vi "FluidtekPrensaCONidentLEDI_v16.vi"() -> ()   [LabVIEW 2026]
uses:
  <vilib>/DAQmx/read.llb/DAQmx Read (Digital 1D Bool NChan 1Samp 1Line).vi
  <vilib>/DAQmx/write.llb/DAQmx Write (Digital 1D Bool NChan 1Samp 1Line).vi
  <vilib>/DAQmx/read.llb/DAQmx Read (Analog 1D Wfm NChan NSamp).vi
  <vilib>/Analysis/baseanly.llb/Mean (DBL).vi
  <vilib>/DAQmx/write.llb/DAQmx Write (Analog DBL 1Chan 1Samp).vi
  <extravilib>/ChannelInstances/Tag-bool/Read With Abort.vi
  <extravilib>/ChannelInstances/Tag-c(dbl,dbl,dbl,dbl,dbl,dbl)/Read With Abort.vi
  <extravilib>/ChannelInstances/Tag-c(dbl,dbl,dbl,dbl,dbl,dbl,dbl,bool,u16)/Write With Abort.vi
  <extravilib>/ChannelInstances/Tag-bool/Write With Abort.vi
  <extravilib>/ChannelInstances/Tag-c(dbl,dbl,dbl,dbl,dbl,dbl,dbl,bool,u16)/Read With Abort.vi
  <extravilib>/ChannelInstances/Tag-c(dbl,dbl,dbl,dbl,dbl,dbl)/Write With Abort.vi
  GlobalesPrensa.vi
  <vilib>/Utility/file.llb/Write Delimited Spreadsheet (DBL).vi
  <vilib>/DAQmx/create/channels.llb/DAQmx Create Channel (AO-Voltage-Basic).vi
  <vilib>/DAQmx/create/channels.llb/DAQmx Create Channel (AI-Voltage-Basic).vi
  <vilib>/DAQmx/configure/timing.llb/DAQmx Timing (Sample Clock).vi
  <vilib>/DAQmx/create/channels.llb/DAQmx Create Channel (DO-Digital Output).vi
  <vilib>/DAQmx/create/channels.llb/DAQmx Create Channel (DI-Digital Input).vi
  <extravilib>/ChannelInstances/Tag-bool/Instantiate.vi
  <extravilib>/ChannelInstances/Tag-bool/Endpoint.vi
  <vilib>/DAQmx/miscellaneous.llb/DAQmx Fill In Error Info.vi
  <extravilib>/ChannelInstances/Tag-c(dbl,dbl,dbl,dbl,dbl,dbl,dbl,bool,u16)/Instantiate.vi
  <extravilib>/ChannelInstances/Tag-c(dbl,dbl,dbl,dbl,dbl,dbl)/Instantiate.vi
  <extravilib>/ChannelInstances/Tag-bool/EndpointRead.vi
  <extravilib>/ChannelInstances/Tag-c(dbl,dbl,dbl,dbl,dbl,dbl)/EndpointRead.vi
  <extravilib>/ChannelInstances/Tag-c(dbl,dbl,dbl,dbl,dbl,dbl,dbl,bool,u16)/Endpoint.vi
  <extravilib>/ChannelInstances/Tag-c(dbl,dbl,dbl,dbl,dbl,dbl,dbl,bool,u16)/EndpointRead.vi
  <extravilib>/ChannelInstances/Tag-c(dbl,dbl,dbl,dbl,dbl,dbl)/Endpoint.vi
  <vilib>/Analysis/NI_AALBase.lvlib
  <extravilib>/ChannelInstances/Tag-bool.lvlib
  <extravilib>/ChannelInstances/Tag-c(dbl,dbl,dbl,dbl,dbl,dbl).lvlib
  <vilib>/ptbypt/NI_PtbyPt.lvlib
  <extravilib>/ChannelInstances/Tag-c(dbl,dbl,dbl,dbl,dbl,dbl,dbl,bool,u16).lvlib
panel:
  out "Archivo":path
  out "Lg log":dbl[](array[numeric])
  in  "PARO DE EMERGENCIA":bool
  out "time/iteration (ms)":u32=210
  in  "Tab Control 3":enum32{"ENSAYO", "REGISTRO"}(tab)
  in  "Tipo ensayos":u16(ring)=1 items=["Flexotraccion en losas", "Tenacidad Vigas"]
  in  "Rampa (mm/min)":dbl=0.1 min=0.0 max=25.0 format="%.3f"
  in  "Rampa (kN/min)":dbl=0.1 min=0.0 max=20.0 format="%.2f"
  in  "Limite fuerza (kN)":dbl=3.0 min=0.0 max=150.0 format="%.2f"
  in  "Limite posicion (mm)":dbl=145.0 min=0.0 max=150.0 format="%.2f"
  in  "Tiempo carga (s)":dbl=3.0 min=0.0 max=300.0 format="%.2g"
  out "Tiempo (s)":dbl format="%.2f"
  in  "Iniciar ensayo":bool
  out "Velocidad norma (mm/min)  2":string="0.05 - 0.1"
  in  "Tenacidad en vigas":u16(ring) items=["ASTM 1609 con100x100x350", "ASTM 1609 con150x150x500", "EFNARC 1996", "VIGAS 14651", "ENS. BARCELONA"]
  in  "Aplicar velocidad de norma":bool
  out "Estado del ensayo":dbl(ring) items=["REPOSO", "CARGA (rampa)", "MANTENIENDO CARGA", "DESCARGA", "RETORNO / FIN", "FALLA - ENSAYO DETENIDO", ""]
  in  "Flexotracción en losas":u16(ring)=3 items=["EFNARC 1996", "EFNARC 1999", "EFNARC 14488-5", "ASTM 1550"]
  out "Velocidad norma (mm/min)":dbl=4.0
  in  "IPAddress QuantumX":string="172.31.236.115"
  out "LicenseIsValid":bool
  in  "Registrar":bool
  in  "ID manual (0=auto)":i32
  in  "Tipo":string
  in  "INFLE":dbl
  in  "Detener registro":bool
  in  "Tab Control 2":T1(tab)
  out "Presión B (bar)":dbl=31.47939829954219 format="%.2f"
  out "Presión A (bar)":dbl=47.7049180327869 format="%.2f"
  out "Vertical Progress Bar":dbl(slide)=3.0
  in  "Tab Control":enum32{"Desplazamiento", "Fuerza"}(tab)
  in  "PID fuerza":T2={"proportional gain (Kc)"=1.0, "integral time (Ti, min)"=0.03, "derivative time (Td, min)"=0.0} {"derivative time (Td, min)" format="%.3f"; "integral time (Ti, min)" format="%.3f"; "proportional gain (Kc)" format="%.3f"}
  out "control signals":dynamicdata(graph)=[{"t0"=timestamp(3594752785.1434503 s since 1904-01-01), "dt"=1.0, "Y"=[3.0]}, {"t0"=timestamp(3594752785.1434503 s since 1904-01-01), "dt"=1.0, "Y"=[3.0680651042487943]}]
  in  "Posicion deseada (mm)":dbl(slide)=3.0 min=2.0 max=150.0 scale format="%#_2f"
  in  "Fuerza deseada (kN)":dbl=0.5 min=0.0 max=150.0 format="%.2f"
  out "Fuerza actual (KN)":dbl format="%.2f"
  out "Posicion actual (mm)":dbl format="%.2f"
  in  "Tipo control":u16(ring) items=["Desplazamiento", "Fuerza"]
  out "fuerza desplazamiento":cluster{dbl[], dbl[]}(graph)
  out "Rigidez estimada (kN/mm)":dbl
  out "Carga maxima (kN)":dbl
  out "Progreso mantenimiento":dbl(slide) scale=0.0..100.0
  out "Tiempo restante carga (s)":dbl
  out "Falla":bool
  out "Causa de la falla":dbl(ring) items=["Sin falla", "CAIDA DE CARGA (rotura)", "SOBRECARGA", "LIMITE DE POSICION", "PARO DE EMERGENCIA", "LIMITE DEL SISTEMA (160 kN)", "SIN LECTURA DE FUERZA (QuantumX)", "LIMITE POR PRESIONES (160 kN)"]
  out "Proteccion de fuerza activa":bool
  in  "Vel. aproximacion (mm/min)":dbl=50.0 min=0.1 max=50.0
  in  "Fmax fuera de ensayo (kN)":dbl=1.0 min=0.2 max=50.0
  out "UPH energizada":bool=TRUE
  out "Nivel tanque":bool
  out "Estado de  filtro":bool=TRUE
  out "Sobrecorriente":bool
  in  "Stop":bool
  out "Estado de motor":bool
  in  "Apagar":bool
  in  "Encender":bool
  in  "Sin proteccion de carga":bool
  out "Consigna posicion interna (mm)":dbl
  out "Parametros avanzados":dbl(ring) items=["POR DEFECTO (bloqueados)", "PERSONALIZADOS (activos)"]
  in  "Codigo acceso":dbl
  in  "Kf lazo fuerza (1/s)":dbl=0.5
  in  "Kx lazo posicion (V/mm)":dbl=30.0
  in  "Ti lazo posicion (s)":dbl=1.5
  # "PB"
  # "PA"
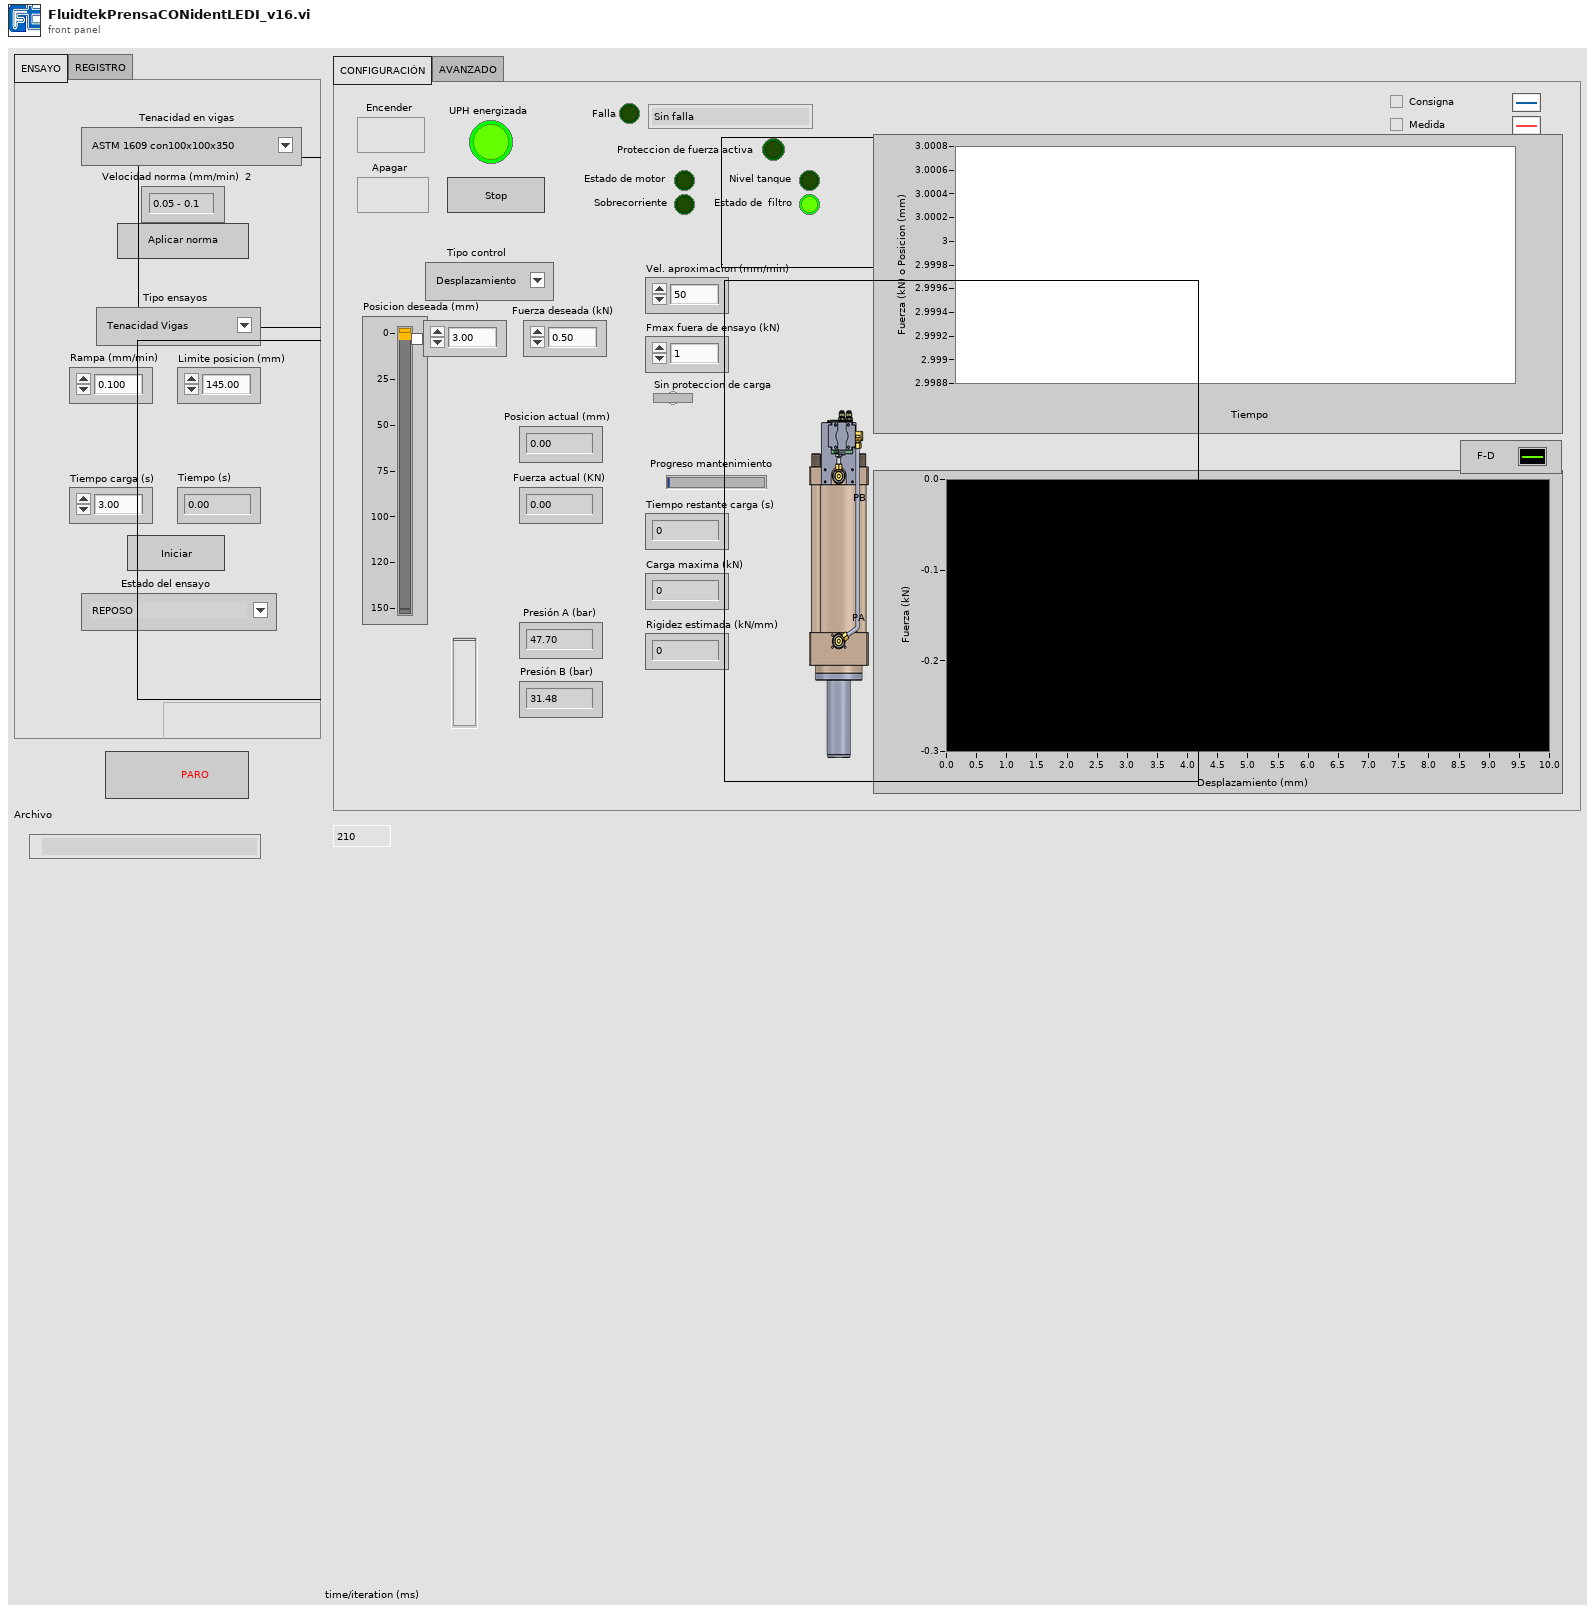
[diagram p1: front panel]
types:
  T1 = enum32{"CONFIGURACIÓN", "AVANZADO", "identificación (no modificar)"}
  T2 = cluster{"proportional gain (Kc)":dbl, "integral time (Ti, min)":dbl, "derivative time (Td, min)":dbl}
  T3 = typedef "Tag-bool.lvlib/))Channel.ctl" = refnum<queue>
  T4 = cluster{"Devices":refnum<k24>[], "Signals":refnum<k24>[]}
  T5 = cluster{"Rampa (mm/min)":dbl, "Rampa (kN/min)":dbl, "Limite posicion (mm)":dbl, "Limite fuerza (kN)":dbl, "Posicion deseada (mm)":dbl, "Fuerza deseada (kN)":dbl, "Tiempo carga (s)":dbl, "Iniciar ensayo":bool, "Tipo control":u16}
  T6 = cluster{"Numeric":dbl, "mean":dbl, "mean":dbl, "mean":dbl, "mean":dbl, "sp":dbl}
  T7 = typedef "Tag-c(dbl,dbl,dbl,dbl,dbl,dbl).lvlib/))Channel.ctl" = refnum<queue>
  T8 = enum8{"Enabled", "Disabled", "Disabled and Grayed Out"}
  T9 = cluster{"Numeric":dbl, dbl, dbl, dbl, dbl, "Limite fuerza (kN)":dbl}
  T10 = typedef "Tag-c(dbl,dbl,dbl,dbl,dbl,dbl,dbl,bool,u16).lvlib/))Channel.ctl" = refnum<queue>
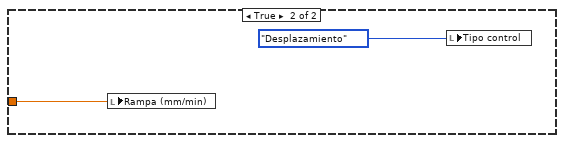
[diagram p5: hidden frame]
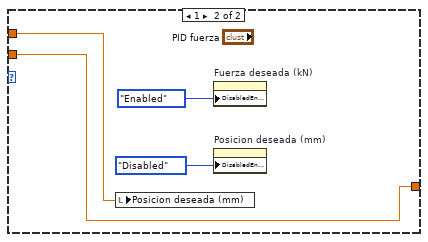
[diagram p6: hidden frame]
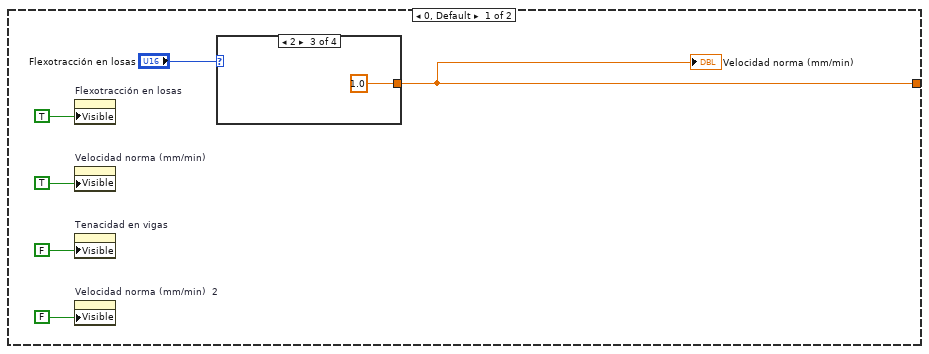
[diagram p7: hidden frame]
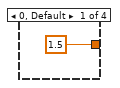
[diagram p8: hidden frame]
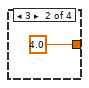
[diagram p9: hidden frame]
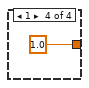
[diagram p10: hidden frame]
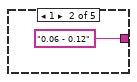
[diagram p11: hidden frame]
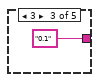
[diagram p12: hidden frame]
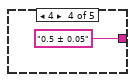
[diagram p13: hidden frame]
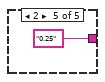
[diagram p14: hidden frame]
diagram:
  w75 = 0 items=["one channel for each line", "one channel for all lines"] ("line grouping")
  w82 = 0 items=["one channel for each line", "one channel for all lines"] ("line grouping")
  w94 = 10348 items=["Volts"=10348, "From Custom Scale"=10065] ("units")
  w97 = -1 items=["Default"=-1, "RSE"=10083, "NRSE"=10078, "Differential"=10106, "Pseudodifferential"=12529] ("input terminal configuration")
  w105 = 10348 items=["Volts"=10348, "From Custom Scale"=10065] ("units")
  w103 = 10106 items=["Default"=-1, "RSE"=10083, "NRSE"=10078, "Differential"=10106, "Pseudodifferential"=12529] ("input terminal configuration")
  w99 = 10123 items=["Finite Samples"=10178, "Continuous Samples"=10123, "Hardware Timed Single Point"=12522] ("sample mode")
  # "Convert device reference to array of device references\n(since ConnectDevice.vi expects an array of devices)..."
  # "Disconnect devices"
  # "Set samplerate and filter frequency for all selected signals."
  # "Initialize HBM Common API for LabVIEW"
  # "End API usage"
  # "Stop DAQ"
  # "Run data acquisition for 10 sec. DAQ-loop: Update signals and do anything with the  measurement values.\n(Here: show first signal in diagram)"
  # "Start DAQ"
  # "Prepare DAQ"
  # "v14: senales [0,1,2,3] -> lazo lee 1,2,3 = W100 (conector 2), Tempsonic (conector 3), Celda via Krenel (conector 4). Filtro 20 Hz, 50 Hz"
  # "Get all signals of the devices"
  # "Connect devices"
  # "Use certain QuantumX device"
  # "Assign the signals...."
  # "Vel. aprox. (mm/min)"
  # "LAZO E/S DIGITAL: encendido/apagado de la unidad hidraulica (contactores), lectura de alarmas (motor, sobrecorriente, nivel, filtro)."
  # "LAZO HMI: lee el panel, habilita/oculta controles segun modo y estado, envia consignas al lazo de control por canal (Tag)."
  # "LAZO DE CONTROL: lectura DAQ (fuerza, desplazamiento, presiones) -> Formula Node 'CONTROLADOR' (maquina de estados + cascada fuerza/posicion + fallas) -> salida servovalvula (AO). Parametros avanzados protegidos con codigo."
  n1 = while {
    tunnel: [w110] -> w3
    tunnel: [w110] -> w2
    tunnel: [w110] -> w1
    i -> [w115]
    stop <- w113 continue-if-true
    n2 = call <vilib>:"DAQmx Reserve Network Device.vi"("device in"=tag "cDAQ9184-1ADC24C", "override reservation?"=TRUE, "error in"=errorcluster {"status"=FALSE, "code"=0, "source"=""}) -> ("error out"=w110:errorcluster)  [unwired: 11 in, 1 out]
    n3 = Unbundle By Name(w110) -> ("status"=w112:bool)
    n4 = Less?(x=w115, y=30) -> (x < y?=w114:bool)
    n5 = And(x=w112, y=w114) -> (x .and. y?=w113:bool)
    n6 = Wait (ms)(milliseconds to wait=u32 2000) -> ()  [unwired: 1 out]
  }
  n7 = call-poly <vilib>:"DAQmx Create Virtual Channel.vi"("lines"=tag "PrensaLEDI_DO/port0/line0:7", "line grouping"=w75, "error in"=w2) -> ("task out"=w76:refnum<k21>, "error out"=w77:errorcluster)  [unwired: 11 in]
  n8 = call-poly <vilib>:"DAQmx Create Virtual Channel.vi"("lines"=tag "PrensaLEDI_DI/port0/line0:7", "line grouping"=w82, "error in"=w3) -> ("task out"=w79:refnum<k21>, "error out"=w80:errorcluster)  [unwired: 11 in]
  n9 = call <vilib>:"DAQmx Start Task.vi"("task/channels in"=w76, "error in"=w77) -> ("task out"=w70:refnum<k21>, "error out"=w69:errorcluster)  [unwired: 12 in]
  n10 = call <vilib>:"DAQmx Start Task.vi"("task/channels in"=w79, "error in"=w80) -> ("task out"=w72:refnum<k21>, "error out"=w71:errorcluster)  [unwired: 12 in]
  n11 = while {
    tunnel: w72 -> [w131]
    tunnel: w71 -> [w130]
    tunnel: [w129] -> w55
    tunnel: [w128] -> w53
    tunnel: w70 -> [w127]
    tunnel: [w126] -> w59
    tunnel: w69 -> [w125]
    tunnel: [w124] -> w57
    tunnel: [w123] -> w6
    stop <- "Stop" stop-if-true
    # "6"
    # "APAGADO Y ENCENDIDO TIPO PULSO"
    # "transmisor de presion"
    # "salida contactor2"
    # "salida al contactor"
    # "pulsador\nemergencia"
    # "GM2"
    n12 = call-poly <vilib>:"DAQmx Read.vi"("task/channels in"=w131, "error in"=w130) -> ("task out"=w129:refnum<k21>, "data"=w146:bool[], "error out"=w128:errorcluster)  [unwired: 11 in]
    n13 = Index Array(array=w146, index=7) -> ()  [unwired: 1 out]
    n14 = global write "GlobalesPrensa.vi" "Salir"("Stop") -> ()
    n15 = Index Array(array=w146, index=5) -> (element=w155:bool)
    "Sobrecorriente" <- w155
    n16 = Index Array(array=w146, index=0) -> (element=w145:bool)
    n17 = Index Array(array=w146, index=2) -> (element=w147:bool)
    n18 = Not(x="Stop") -> (.not. x?=w144:bool)
    n19 = Not(x=w147) -> (.not. x?=→"Estado de  filtro":bool)
    n20 = Not(x=w155) -> (.not. x?=→"UPH energizada":bool)
    n21 = And(x=w145, y=w144) -> (x .and. y?=w151:bool)
    n22 = Index Array(array=w146, index=1) -> (element=→"Nivel tanque":bool)
    n23 = local read "PARO DE EMERGENCIA"() -> (w120:bool)
    n24 = Not(x=w151) -> (.not. x?=w152:bool)
    n25 = Not(x=w151) -> (.not. x?=w153:bool)
    n26 = Or(x="Apagar", y=w152) -> (x .or. y?=w121:bool)
    n27 = Or(x=w121, y=w120) -> (x .or. y?=w122:bool)
    n28 = while {
      shift-right: [w159] -> w156
      shift-left: _ -> [w161]
      tunnel: "Encender" -> [w160]
      tunnel: w122 -> [w158]
      stop <- FALSE continue-if-true
      n29 = Exclusive Or(1:w158, 2:w160) -> (0:w162:bool)
      n30 = Select(t=w160, s=w162, f=w161) -> (s? t:f=w159:bool)
    }
    "Estado de motor" <- w156
    n31 = Wait (ms)(milliseconds to wait=u32 500) -> ()  [unwired: 1 out]
    n32 = Replace Array Subset(array=bool[] [FALSE, FALSE, FALSE, FALSE, FALSE, FALSE, FALSE, FALSE], new element #1=w156, index #1=0 ("index"), new element #2=w153, index #2=2 ("index"), new element #3=TRUE ("new element/subarray"), index #3=5 ("index")) -> (w154:bool[])
    n33 = call-poly <vilib>:"DAQmx Write.vi"("task/channels in"=w127, "data"=w154, "error in"=w125) -> ("task out"=w126:refnum<k21>, "error out"=w124:errorcluster)  [unwired: 10 in, 1 out]
    n34 = call <extravilib>:"Write.vi"("element"="Stop") -> ("channel"=w123:T3)  [unwired: 1 out]
  }
  n35 = call-poly <vilib>:"DAQmx Create Virtual Channel.vi"("maximum value"=10.0, "minimum value"=0.0, "input terminal configuration"=w103, "physical channels"=tag "PrensaLEDI_AI/ai0:3", "units"=w105, "error in"=w1) -> ("task out"=w106:refnum<k21>, "error out"=w107:errorcluster)  [unwired: 8 in]
  n36 = call-poly <vilib>:"DAQmx Create Virtual Channel.vi"("maximum value"=10.0, "minimum value"=-10.0, "output terminal configuration"=w97, "physical channels"=tag "PrensaLEDI_AO/ao0", "units"=w94, "error in"=w1) -> ("task out"=w98:refnum<k21>, "error out"=w96:errorcluster)  [unwired: 8 in]
  n37 = call-poly <vilib>:"DAQmx Timing.vi"("task/channels in"=w106, "sample mode"=w99, "samples per channel"=500000, "rate"=200000.0, "error in"=w107) -> ("task out"=w67:refnum<k21>, "error out"=w66:errorcluster)  [unwired: 9 in]
  n38 = call <vilib>:"DAQmx Start Task.vi"("task/channels in"=w67, "error in"=w66) -> ("task out"=w65:refnum<k21>, "error out"=w64:errorcluster)  [unwired: 12 in]
  n39 = call <vilib>:"DAQmx Start Task.vi"("task/channels in"=w98, "error in"=w96) -> ("task out"=w87:refnum<k21>, "error out"=w86:errorcluster)  [unwired: 12 in]
  n40 = feedback-in #1(w6) -> ()
  n41 = feedback #1() -> ()  [unwired: 2 in]
  n42 = call <vilib>:"DAQmx Stop Task.vi"("task/channels in"=w59, "error in"=w57) -> ("task out"=w58:refnum<k21>, "error out"=w56:errorcluster)  [unwired: 12 in]
  n43 = call <vilib>:"DAQmx Stop Task.vi"("task/channels in"=w55, "error in"=w53) -> ("task out"=w54:refnum<k21>, "error out"=w52:errorcluster)  [unwired: 12 in]
  n44 = call <vilib>:"DAQmx Clear Task.vi"("task in"=w58, "error in"=w56) -> ("error out"=w74:errorcluster)  [unwired: 13 in]
  n45 = call <vilib>:"DAQmx Clear Task.vi"("task in"=w54, "error in"=w52) -> ("error out"=w73:errorcluster)  [unwired: 13 in]
  n46 = call <vilib>:"Simple Error Handler.vi"("error in (no error)"=w74) -> ()  [unwired: 4 in, 5 out]
  n47 = call <vilib>:"Simple Error Handler.vi"("error in (no error)"=w73) -> ()  [unwired: 4 in, 5 out]
  n48 = call <userlib>:"Init.vi"() -> ("LicenseIsValid"=→"LicenseIsValid":bool, "Error out"=w13:errorcluster)  [unwired: 8 in, 1 out]
  n49 = call <userlib>:"QuantumX_Device.vi"("Error in"=w13, "IPAddress"="IPAddress QuantumX") -> ("Error out"=w14:errorcluster, "Device"=w11:refnum<k24>)  [unwired: 6 in]
  n50 = Build Array(w11) -> (w10:refnum<k24>[])
  n51 = call <userlib>:"ConnectDevice.vi"("Error in"=w14, "Devices"=w10) -> ("Error out"=w36:errorcluster, "Devices"=w35:refnum<k24>[])  [unwired: 7 in, 1 out]
  n52 = call <userlib>:"GetSignals.vi"("Error in"=w36, "Devices"=w35) -> ("Error out"=w30:errorcluster, "DevicesAndSignals"=w31:T4)  [unwired: 8 in]
  n53 = Unbundle By Name(w31) -> ("Devices"=w24:refnum<k24>[], "Signals"=w28:refnum<k24>[])
  n54 = Index Array(array=w28, index #1=0 ("Index"), index #2=1 ("Index"), index #3=2 ("Index"), index #4=3 ("Index")) -> (element #1=w27:refnum<k24>, element #2=w26:refnum<k24>, element #3=w19:refnum<k24>, element #4=w18:refnum<k24>)
  n55 = Build Array(w27, w26, w19, w18) -> (w25:refnum<k24>[])
  n56 = Bundle(cluster=w31, "Devices"=w24, "Signals"=w25) -> (w32:T4)
  n57 = Unbundle By Name(w32) -> ("Signals"=w48:refnum<k24>[])
  n58 = case shown="No Error" w30 {
    tunnel: w30 -> [w168 w174]
    tunnel: w48 -> [w167 _]
    tunnel: [w166 w174] -> w47
    frame No Error {
      # "Filter frequency:"
      # "Samplerate:"
      n59 = for {
        tunnel: w168 -> [w173]
        tunnel: 50.0 ("SampleRate") -> [w172]
        tunnel: 20.0 ("FilterFrequency") -> [w171]
        tunnel: w167 -> [w170] mode=indexing
        tunnel: [w169] -> w166
        stop <- w169 stop-if-true
        n60 = call <userlib>:"ConfigSignal.vi"("Error in"=w173, "SampleRate"=w172, "FilterFrequency"=w171, "Signal"=w170) -> ("Error out"=w169:errorcluster)  [unwired: 7 in]
      }
    }
    frame Error {
    }
  }
  n61 = call <userlib>:"AssignSignals.vi"("Error in"=w47, "DevicesAndSignals"=w32) -> ("Error out"=w45:errorcluster, "DevicesAndSignals"=w46:T4)  [unwired: 8 in]
  n62 = call <userlib>:"PrepareDAQ.vi"("Error in"=w45, "DevicesAndSignals"=w46) -> ("Error out"=w42:errorcluster, "DaqMeasurement"=w43:refnum<k24>, "DevicesAndSignals"=w44:T4)  [unwired: 7 in]
  n63 = call <userlib>:"StartDaq.vi"("DevicesAndSignals"=w44, "DaqMeasurement"=w43, "AcquisitionMode"=2, "Error in"=w42) -> ("DevicesAndSignals"=w39:T4, "DaqMeasurement"=w40:refnum<k24>, "Error out"=w41:errorcluster)  [unwired: 7 in, 2 out]
  n64 = while {
    tunnel: w40 -> [w235]
    tunnel: w39 -> [w234]
    tunnel: [w230] -> w38
    tunnel: [w229] -> w37
    tunnel: w41 -> [w236]
    tunnel: [w228] -> w5
    shift-right: [w196] -> _
    shift-left: 0 -> [w221]
    shift-right: [w187] -> _
    shift-left: FALSE ("Registrar") -> [w192]
    shift-right: [w191] -> _
    shift-left: _ -> [w193]
    stop <- w182 stop-if-true
    n65 = global read "GlobalesPrensa.vi" "Salir"() -> (w181:bool)
    n66 = Get Date/Time In Seconds() -> (seconds since 1Jan1904=w204:timestamp)
    n67 = Format Into String(format string="D:\\\\%<%Y>T\\\\%03d-%<%Y>T", w204, "INFLE", w204) -> (resulting string=w206:string)  [unwired: 2 in, 1 out]
    n68 = Or(x=w181, y="Detener registro") -> (x .or. y?=w182:bool)
    n69 = String To Path(string=w206) -> (path=w209:path)
    n70 = Create Folder(path (use dialog)=w209) -> (error out=w207:errorcluster)  [unwired: 2 in, 2 out]
    n71 = Format Into String(format string="%s P*", "Tipo") -> (resulting string=w210:string)  [unwired: 2 in, 1 out]
    n72 = call <vilib>:"Clear Errors.vi"("error in (no error)"=w207) -> ("error out"=w208:errorcluster)  [unwired: 5 in, 1 out]
    n73 = List Folder(path=w209, pattern=w210, error in=w208) -> (path out=w219:path, filenames=w211:string[])  [unwired: 1 in, 2 out]
    n74 = Not(x=w192) -> (.not. x?=w198:bool)
    n75 = for {
      tunnel: w211 -> [w263] mode=indexing
      tunnel: [w261] -> w212 mode=indexing
      n76 = Scan From String(format string="%s P%d", input string=w263) -> (error out=w260:errorcluster, output 2=w261:i32)  [unwired: 5 in, 2 out]
      n77 = call <vilib>:"Clear Errors.vi"("error in (no error)"=w260) -> ()  [unwired: 5 in, 2 out]
    }
    n78 = Array Max & Min(array=w212) -> (max value=w213:i32)  [unwired: 3 out]
    n79 = Greater Than 0?(x="ID manual (0=auto)") -> (x > 0?=w215:bool)
    n80 = Increment(x=w213) -> (x+1=w214:i32)
    n81 = Select(t="ID manual (0=auto)", s=w215, f=w214) -> (s? t:f=w217:i32)
    n82 = global read "GlobalesPrensa.vi" "Ensayando"() -> (w188:bool)
    n83 = global read "GlobalesPrensa.vi" "InfoEnsayo"() -> (w185:string)
    n84 = Format Into String(format string="%s P%d.csv", "Tipo", w217) -> (resulting string=w218:string)  [unwired: 2 in, 1 out]
    n85 = Or(x="Registrar", y=w188) -> (x .or. y?=w187:bool)
    n86 = Build Path(base path=w219, name or relative path=w218) -> (appended path=w194:path)
    n87 = Get Date/Time In Seconds() -> (seconds since 1Jan1904=w186:timestamp)
    n88 = And(x=w187, y=w198) -> (x .and. y?=w199:bool)
    n89 = Select(t=w193, s=w192, f=w194) -> (s? t:f=w191:path)
    "Archivo" <- w191
    n90 = Format Into String(format string="Fecha\t%<%Y-%m-%d %H:%M:%S>T\nNorma\t%s\nFrecuencia (Hz)\t50\nRunning Time\tDeflection\tDisplacement\tLoad\ns\tmm\tmm\tkN\n", w186, w185) -> (resulting string=w184:string)  [unwired: 2 in, 1 out]
    n91 = case shown="True" w199 {
      tunnel: [_ w258] -> w200
      tunnel: w191 -> [_ w256]
      tunnel: w184 -> [_ w257]
      frame False {
      }
      frame True {
        (unwired) "" ("text")
        (unwired) errorcluster {"status"=FALSE, "code"=0, "source"=""} ("error in")
        (unwired) "" ("prompt (Choose or enter file path)")
        # "t (s)\\testado\\tconsigna\\tF (kN)\\tx (mm)\\txsp (mm)\\tu (V)\\tkh (kN/mm)\\tdt (s)\\tfalla\\tcausa\\tprot\\n"
        n92 = Path To String(path=w256) -> (string=w255:string)
        n93 = Search and Replace String(replace all?=FALSE ("replace all? (F)"), case sensitive?=FALSE ("ignore case? (F)"), input string=w255, search string=".csv", replace string="_control.csv" ("replace string (\"\")"), offset=0 ("offset (0)"), error in=errorcluster {"status"=FALSE, "code"=0, "source"=""} ("error in (no error)")) -> (result string=w248:string)  [unwired: 1 in, 3 out]
        n94 = String To Path(string=w248) -> (path=w247:path)
        n95 = Write to Text File(file (use dialog)=w247, text="t (s)\testado\tconsigna\tF (kN)\tx (mm)\txsp (mm)\tu (V)\tkh (kN/mm)\tdt (s)\tfalla\tcausa\tprot\tpA (bar)\tpB (bar)\tFp (kN)\n") -> (error out=w245:errorcluster)  [unwired: 2 in, 2 out]
        n96 = flat-sequence {
          tunnel: w247 -> [w259]
          tunnel: w245 -> [_]
          frame #0 {
            n97 = global write "GlobalesPrensa.vi" "ArchivoControl"(w259) -> ()
          }
        }
        n98 = Write to Text File(file (use dialog)=w256, text=w257) -> (error out=w258:errorcluster)  [unwired: 2 in, 2 out]
      }
    }
    n99 = call <userlib>:"UpdateMeasurementValues.vi"("Error in"=w236, "DaqMeasurement"=w235, "DevicesAndSignals"=w234) -> ("Error out"=w231:errorcluster, "DaqMeasurement"=w232:refnum<k24>, "DevicesAndSignals"=w233:T4)  [unwired: 6 in]
    n100 = for {
      N: 3 -> [_]
      shift-right: [w275] -> w229
      shift-left: w233 -> [w279]
      shift-right: [w276] -> w230
      shift-left: w232 -> [w278]
      shift-right: [w274] -> w228
      shift-left: w231 -> [w277]
      tunnel: [w269] -> w180 mode=indexing
      i -> [w272]
      n101 = Add(x=w272, y=1.0) -> (x+y=w271:dbl)
      n102 = call <userlib>:"GetMeasurementValues.vi"("Error in"=w277, "Index"=w271, "DaqMeasurement"=w278, "DevicesAndSignals"=w279) -> ("Error out"=w274:errorcluster, "Waveform"=w270:waveform(dbl), "DaqMeasurement"=w276:refnum<k24>, "DevicesAndSignals"=w275:T4)  [unwired: 2 in, 2 out]
      n103 = Unbundle By Name(w270) -> ("Y"=w269:dbl[])
    }
    n104 = feedback #2() -> (w178:dbl)  [unwired: 1 in]
    n105 = Tick Count (ms)() -> (millisecond timer value=w179:u32)
    n106 = Array Size(array=w180) -> (size(s)=w224:i32[])
    n107 = Index Array(array=w224, index=1) -> (element=w222:i32)
    n108 = for {
      N: w222 -> [_]
      tunnel: [w266] -> w220 mode=indexing
      tunnel: w221 -> [w264]
      i -> [w268]
      n109 = Add(x=w268, y=w264) -> (x+y=w267:i32)
      n110 = Multiply(x=w267, y=0.02) -> (x*y=w266:dbl)
    }
    n111 = Add(x=w221, y=w222) -> (x+y=w197:i32)
    n112 = feedback #3() -> (w177:dbl)  [unwired: 1 in]
    n113 = formula code="int32 n,m; m=sizeOfDim(D,0); n=sizeOfDim(D,1);\nif (m>2 && n>0) { Fq=D[2][n-1]; tq=tk; } else { Fq=Fo; tq=to; }"("D"=w180, "tk"=w179, "Fo"=w178, "to"=w177) -> ("Fq"=w176:dbl, "tq"=w175:dbl)
    n114 = feedback-in #2(w176) -> ()
    n115 = global write "GlobalesPrensa.vi" "F_QX"(w176) -> ()
    n116 = global write "GlobalesPrensa.vi" "tQX"(w175) -> ()
    n117 = feedback-in #3(w175) -> ()
    n118 = Select(t=w197, s=w187, f=0) -> (s? t:f=w196:i32)
    n119 = case shown="True" w187 {
      tunnel: w180 -> [_ w244]
      tunnel: w220 -> [_ w243]
      tunnel: w200 -> [_ w238]
      tunnel: w191 -> [_ w237]
      frame False {
      }
      frame True {
        n120 = Insert Into Array(array=w244, index (row)=0, new element=w243) -> (w241:dbl[][])  [unwired: 1 in]
        n121 = call-poly <vilib>:"Write Delimited Spreadsheet.vi"("file path (dialog if empty)"=w237, "2D data"=w241, "append to file? (new file:F)"=TRUE, "error in (no error)"=w238, "transpose? (no:F)"=TRUE) -> ()  [unwired: 9 in, 2 out]
      }
    }
    n122 = Wait Until Next ms Multiple(millisecond multiple=u32 20 ("Vielfache von ms")) -> ()  [unwired: 1 out]
  }
  n123 = call <vilib>:"Clear Errors.vi"("error in (no error)"=w5) -> ("error out"=w4:errorcluster)  [unwired: 5 in, 1 out]
  n124 = call <userlib>:"StopDaq.vi"("Error in"=w4, "DaqMeasurement"=w38, "DevicesAndSignals"=w37) -> ("Error out"=w17:errorcluster, "DevicesAndSignals"=w16:T4)  [unwired: 7 in]
  n125 = call <userlib>:"DisconnectDevice.vi"("Error in"=w17, "DevicesAndSignals"=w16) -> ("Error out"=w15:errorcluster)  [unwired: 9 in]
  n126 = call <vilib>:"Simple Error Handler.vi"("error in (no error)"=w15) -> ("error out"=w34:errorcluster)  [unwired: 4 in, 4 out]
  n127 = call <userlib>:"DisposeApi.vi"("Error in"=w34) -> ()  [unwired: 10 in, 1 out]
  n128 = global write "GlobalesPrensa.vi" "Salir"(FALSE ("Salir")) -> ()
  n129 = while {
    tunnel: w65 -> [w370]
    tunnel: w64 -> [w369]
    tunnel: [w368] -> w63
    tunnel: [w367] -> w61
    tunnel: [w366] -> w89
    tunnel: [w365] -> w88
    tunnel: w87 -> [w364]
    tunnel: w86 -> [w363]
    shift-right: [w350] -> _
    shift-left: u32[] [] -> [w351]
    tunnel: w51 -> [w341]
    tunnel: [w349] -> w68
    tunnel: w6 -> [w347]
    stop <- w348 stop-if-true
    # "bar"
    # "volt"
    # "bar"
    # "volt"
    # "embolo"
    n130 = call <extravilib>:"Read.vi"("channel"=w341) -> ("element"=w282:T5)  [unwired: 1 in, 1 out]
    n131 = call <extravilib>:"Read.vi"("channel"=w347) -> ("element"=w348:bool)  [unwired: 1 in, 1 out]
    n132 = Tick Count (ms)() -> (millisecond timer value=w353:u32)
    n133 = feedback #4(w353) -> (w354:u32)
    n134 = feedback-in #4(w353) -> ()
    n135 = call-poly <vilib>:"DAQmx Read.vi"("task/channels in"=w370, "number of samples per channel"=4000, "error in"=w369) -> ("task out"=w368:refnum<k21>, "data"=w362:waveform(dbl)[], "error out"=w367:errorcluster)  [unwired: 10 in]
    n136 = Subtract(x=w353, y=w354) -> (x-y=w352:u32)
    "time/iteration (ms)" <- w352
    n137 = Split Signals(w362) -> (w358:dynamicdata, w361:dynamicdata, w360:dynamicdata, w359:dynamicdata)  [unwired: 4 in]
    n138 = call "Convert from Dynamic Data3"("Dynamic Data Type"=w360) -> ("Array"=w337:dbl[])  [unwired: 3 in]
    n139 = call "Convert from Dynamic Data4"("Dynamic Data Type"=w359) -> ("Array"=w336:dbl[])  [unwired: 3 in]
    n140 = call "Convert from Dynamic Data"("Dynamic Data Type"=w358) -> ("Array"=w339:dbl[])  [unwired: 3 in]
    n141 = call "Convert from Dynamic Data2"("Dynamic Data Type"=w361) -> ("Array"=w338:dbl[])  [unwired: 3 in]
    n142 = Build Array (concatenate)(w351, w352) -> (w350:u32[])
    n143 = call-poly <vilib>:"Mean.vi"("X"=w337) -> ("mean"=w288:dbl)  [unwired: 1 out]
    n144 = call-poly <vilib>:"Mean.vi"("X"=w336) -> ("mean"=w287:dbl)  [unwired: 1 out]
    n145 = call-poly <vilib>:"Mean.vi"("X"=w339) -> ("mean"=w286:dbl)  [unwired: 1 out]
    n146 = call-poly <vilib>:"Mean.vi"("X"=w338) -> ("mean"=w284:dbl)  [unwired: 1 out]
    n147 = expression code="15*x"(w286) -> (w285:dbl)
    n148 = expression code="20*x"(w284) -> (w283:dbl)
    n149 = Unbundle By Name(w282) -> ("Rampa (mm/min)"=w346:dbl, "Rampa (kN/min)"=w345:dbl, "Limite posicion (mm)"=w316:dbl, "Limite fuerza (kN)"=w344:dbl, "Posicion deseada (mm)"=w343:dbl, "Fuerza deseada (kN)"=w342:dbl, "Tiempo carga (s)"=w323:dbl, "Iniciar ensayo"=w335:bool, "Tipo control"=w317:u16)
    n150 = case shown="1" w317 {
      tunnel: w346 -> [w382 _]
      tunnel: w343 -> [w381 _]
      tunnel: w342 -> [_ w384]
      tunnel: w345 -> [_ w385]
      tunnel: [w382 w385] -> w325
      tunnel: [w381 w384] -> w321
      tunnel: [w380 w383] -> w326
      tunnel: w316 -> [w380 _]
      tunnel: w344 -> [_ w383]
      frame 0, Default {
      }
      frame 1 {
      }
    }
    n151 = Select(t=10.0, s=w335, f=0.0) -> (s? t:f=w327:dbl)
    n152 = call "TIME.vi"("Numeric 2"=0, "y"=w327) -> ("Numeric"=w322:dbl)
    n153 = expression code="(x-1.9826)*12.5"(w288) -> (w281:dbl)
    n154 = expression code="(x-1.9682)*50"(w287) -> (w280:dbl)
    n155 = formula code="/* ===========================================================================\n   PARAMETROS DEL CONTROLADOR  ->  arreglo P[8] que consume PID.c\n   Formula Node \"ParamPID\". Es el UNICO lugar donde estan los valores por\n   defecto: PID.c no los repite (si P no llega completo, PID.c da FALLA y 0 V).\n   ===========================================================================\n\n   TERMINALES\n     Entradas  cod   codigo de acceso (2026 habilita los valores del panel)\n               Kx    ganancia del lazo de posicion [V/mm]\n               Tix   tiempo integral del lazo de posicion [s]\n               Kf    correccion del lazo de fuerza [1/s]\n     Salidas   P     arreglo de 8 parametros (el que lee PID.c)\n               act   1 = se usan los valores del panel, 0 = valores por defecto\n\n   P[]      significado                                 defecto   rango del panel\n     P[0]   Kx   ganancia PI de posicion [V/mm]           30        1 ... 100\n     P[1]   Tix  tiempo integral [s]                      1.5       0.1 ... 60\n     P[2]   Kf   correccion del lazo de fuerza [1/s]      0.5       0.05 ... 5\n     P[3]   rigidez inicial estimada [kN/mm]              1         (fijo)\n     P[4]   caida de carga que dispara FALLA (fraccion del pico)   0.3   (fijo)\n     P[5]   sobrecarga que dispara FALLA (fraccion de lim)         1.2   (fijo)\n     P[6]   velocidad de retorno [mm/min], todos los casos y modos 50    (fijo)\n     P[7]   variacion maxima de la salida u [V/s]         40        (fijo)\n   =========================================================================== */\n\nfloat64 P[8];\n\n/* valores por defecto */\nP[0] = 30;\nP[1] = 1.5;\nP[2] = 0.5;\nP[3] = 1;\nP[4] = 0.3;\nP[5] = 1.2;\nP[6] = 50;\nP[7] = 40;\nact = 0;\n\n/* con el codigo de acceso, los tres primeros salen del panel, limitados a rangos seguros */\nif (cod==2026) {\n    P[0] = max(1,min(100,Kx));\n    P[1] = max(0.1,min(60,Tix));\n    P[2] = max(0.05,min(5,Kf));\n    act = 1;\n}"("cod"="Codigo acceso", "Kx"="Kx lazo posicion (V/mm)", "Tix"="Ti lazo posicion (s)", "Kf"="Kf lazo fuerza (1/s)") -> ("P"=w312:dbl[], "act"=→"Parametros avanzados":dbl)
    n156 = Boolean To (0,1)(Boolean="PARO DE EMERGENCIA") -> (0, 1=w302:i16)
    n157 = Boolean To (0,1)(Boolean="Sin proteccion de carga") -> (0, 1=w289:i16)
    n158 = feedback #5() -> (w318:dbl[])  [unwired: 1 in]
    n159 = call <vilib>:"High Resolution Relative Seconds.vi"() -> ("relative seconds"=w295:dbl)
    n160 = feedback #6() -> (w324:dbl)  [unwired: 1 in]
    n161 = feedback #7() -> (w328:dbl)  [unwired: 1 in]
    n162 = feedback #8() -> (w332:dbl)  [unwired: 1 in]
    n163 = feedback #9() -> (w330:dbl)  [unwired: 1 in]
    n164 = formula code="/* ===========================================================================\n   CONTROLADOR PRENSA FLUIDTEK v17 - cascada fuerza -> posicion\n   Formula Node de FluidtekPrensaCONidentLEDI_v16.vi  (un paso del lazo, ~20 ms)\n   ===========================================================================\n\n   QUE HACE\n     1. Genera la consigna sp segun el estado st (maquina de estados).\n     2. Lazo externo: convierte sp (posicion o fuerza) en consigna de posicion\n        x_ref. En fuerza se divide por la rigidez estimada rig [kN/mm].\n     3. Lazo interno: PI de posicion -> comando u [V] a la servovalvula.\n     4. Protecciones: celda (F_corte), sobrecarga, caida de carga, limite de\n        posicion, paro de emergencia, presiones (desactivado) y NaN.\n\n   ESTADOS  st      0 reposo/aproximacion   1 carga   2 mantener   3 descarga\n                    4 retorno/fin           5 FALLA\n   CAUSAS   causa   0 ninguna  1 caida de carga  2 sobrecarga  3 limite de posicion\n                    4 paro de emergencia  5 limite de la celda (F_corte)\n                    7 limite por presiones (pa >= pa_max o F_pres >= F_corte)\n   MODOS    modo    0 control de desplazamiento [mm]    1 control de fuerza [kN]\n\n   TERMINALES (el nombre es el del terminal en la VI)\n     Entradas  x        posicion del vastago [mm]\n               F        fuerza de la celda [kN]\n               modo     ver arriba\n               t, tr    tiempo del ensayo [s] y reloj de alta resolucion [s]\n               pa       presion camara A, SIN vastago [bar]  (TR44.2, ai2)\n               pb       presion camara B, CON vastago [bar]  (TR49.2, ai3)\n                        (llegan en bar reales; el escalado esta en el diagrama:\n                         pa = (V_ai2 - 1.9826)*12.5   pb = (V_ai3 - 1.9682)*50)\n               vjog     velocidad de aproximacion fuera de ensayo [mm/min]\n               Flib     limite de fuerza fuera de ensayo [kN]\n               sinprot  1 = sin proteccion de carga fuera de ensayo\n               ini      INICIAR (>= 5 activo)      inip   valor anterior de ini\n               spm      consigna manual fuera de ensayo [mm o kN]\n               lim      consigna final del ensayo  rate   rampa [unidad/min]\n               tc       tiempo de mantenimiento [s]   xlim limite de posicion [mm]\n               paro     paro de emergencia\n               stp, f0p, tsp   st, f0 y ts del paso anterior\n               P        parametros avanzados (arreglo, >= 8)\n               S        estado persistente (arreglo de 12)\n               tkq, tqx SIN USO (vigilancia del QuantumX, retirada en v16)\n     Salidas   st, f0, ts, inio, sp, prot, prog, trest, falla, causa,\n               Fpko, xspo, kho, u, So (estado, 12), Lg (registro, 15)\n\n   PARAMETROS P[]  los entrega el Formula Node ParamPID (ParamPID.c), que es el\n                   unico lugar con valores por defecto y rangos. Si P trae menos de\n                   8 elementos el paso termina en FALLA con u = 0 (seccion 12).\n     P[0] Kx  ganancia del PI de posicion [V/mm]    P[1] Tix tiempo integral [s]\n     P[2] Kf  correccion del lazo de fuerza [1/s]   P[3] rigidez inicial [kN/mm]\n     P[4] caida de carga que dispara FALLA 1, fraccion del pico\n     P[5] sobrecarga que dispara FALLA 2, fraccion de lim\n     P[6] velocidad de retorno [mm/min]             P[7] variacion maxima de u [V/s]\n\n   ESTADO PERSISTENTE S[] -> So[]  (llega como 12 ceros en la primera iteracion)\n     0 x_ref  1 rig   2 F_pico   3 integ   4 sp_prev   5 t_prev\n     6 F_ref  7 x_ref_rig  8 x_inicio  9 u_prev  10 modo_prev  11 causa_act\n\n   REGISTRO Lg[]\n     0 t  1 st  2 sp  3 F  4 x  5 x_ref  6 u  7 rig  8 dt  9 falla  10 causa\n     11 prot  12 pa  13 pb  14 F_pres\n\n   PARO: salida 0 V, controlador en seguimiento (sin salto al soltarlo).\n   El historial de versiones esta en git (git log -- labview_control_software/PID.c).\n   v16: misma logica que v15, verificada paso a paso con 320 000+ pasos\n        aleatorios; solo cambian nombres, orden de la cabecera y se retira el\n        codigo muerto del QuantumX (causa 6).\n   v17: los valores por defecto de P viven solo en ParamPID.c; si P llega\n        incompleto ya no se inventan defaults: FALLA con u = 0.\n   =========================================================================== */\n\n\n/* ---------------------------------------------------------------------------\n   0. DECLARACIONES Y CONSTANTES\n   (el Formula Node no tiene #define: las constantes son variables)\n   --------------------------------------------------------------------------- */\n\n/* parametros de P */\nfloat64 Kx, Tix, Kf, rig_ini, frac_caida, frac_sobre, v_retorno, du_max, par_ok;\n/* estado persistente (S) */\nfloat64 x_ref, rig, F_pico, integ, sp_prev, t_prev, F_ref, x_ref_rig, x_inicio;\nfloat64 u_prev, modo_prev, causa_act;\n/* variables de trabajo */\nfloat64 med, dt, v_aprox, F_lib;\nfloat64 dif, vel_sp, paso_sp, dF_min, rig_nueva;\nfloat64 x_ref_ini, x_ref_prev, err, u_pi;\nfloat64 F_pres, lim_pres;\n/* arreglos de salida */\nfloat64 So[12];\nfloat64 Lg[15];\n/* constantes de seguridad y de ajuste */\nfloat64 F_corte, pa_max, prot_pres_on, v_des, u_max, x_win, v_lenta;\nfloat64 rig_min, rig_max, alfa_rig, frac_freno, frac_pico_min, margen_xlim;\nfloat64 dF_min_rig, dx_min_rig, dx_sin_contacto;\nfloat64 cFpA, cFpB;\n/* codigos de estado y de causa */\nfloat64 ST_REPOSO, ST_CARGA, ST_MANTIENE, ST_DESCARGA, ST_RETORNO, ST_FALLA;\nfloat64 CAU_NINGUNA, CAU_CAIDA, CAU_SOBRECARGA, CAU_LIM_POS, CAU_PARO, CAU_FCORTE, CAU_PRESION;\n\nF_corte  = 160;     /* kN: corte por la celda. 160 kN ~ 80 bar con el cilindro 160/80: BAJAR (CLAUDE.md 6) */\npa_max   = 95;      /* bar: corte por presion de la camara A (el TR44.2 satura a 100 bar) */\nprot_pres_on = 0;   /* 0 = corte por presiones DESACTIVADO (desde 2026-11-03); 1 = activo */\nv_des    = 40;      /* kN/min: carga/descarga en fuerza fuera de ensayo y descarga en ensayo */\nu_max    = 10;      /* V: saturacion del comando (tambien umbral del anti-windup) */\nx_win    = 2;       /* mm: x_ref no se separa de x mas que esto */\nv_lenta  = 2;       /* mm/min: avance lento fuera de ensayo con compresion */\nrig_min  = 0.02;    /* kN/mm: rigidez estimada minima */\nrig_max  = 50;      /* kN/mm: rigidez estimada maxima */\nalfa_rig = 0.3;     /* filtro de la rigidez estimada */\nfrac_freno    = 0.25;   /* avance lento si F > frac_freno*F_lib (fuera de ensayo) */\nfrac_pico_min = 0.2;    /* la caida de carga solo cuenta si el pico fue > 20 % de lim */\nmargen_xlim   = 0.5;    /* mm: tolerancia sobre el limite de posicion xlim */\ndF_min_rig      = 0.05; /* kN: cambio minimo de fuerza para actualizar la rigidez */\ndx_min_rig      = 0.002;/* mm: cambio minimo de posicion para actualizar la rigidez */\ndx_sin_contacto = 5;    /* mm: mas que esto sin cambio de F = sin contacto */\n\n/* Fp = A_A*pa - A_B*pb con el cilindro 160/80 mm (kN/bar = A[m2]*100):\n   A_A = 201.06 cm2 (camara A, sin vastago), A_B = 150.80 cm2 (camara B, con vastago) */\ncFpA = 2.0106;\ncFpB = 1.5080;\n\nST_REPOSO = 0;  ST_CARGA = 1;  ST_MANTIENE = 2;  ST_DESCARGA = 3;  ST_RETORNO = 4;  ST_FALLA = 5;\nCAU_NINGUNA = 0;  CAU_CAIDA = 1;  CAU_SOBRECARGA = 2;  CAU_LIM_POS = 3;\nCAU_PARO = 4;  CAU_FCORTE = 5;  CAU_PRESION = 7;\n\n/* parametros de ParamPID. Si P llega incompleto los valores son inertes y la\n   seccion 12 deja el paso en FALLA con u = 0 */\npar_ok = sizeOfDim(P,0)>=8;\nKx=0; Tix=1; Kf=0; rig_ini=1; frac_caida=1; frac_sobre=1; v_retorno=0; du_max=0;\nif (par_ok) {\n    Kx=P[0]; Tix=P[1]; Kf=P[2]; rig_ini=P[3];\n    frac_caida=P[4]; frac_sobre=P[5]; v_retorno=P[6]; du_max=P[7];\n}\n\n/* ---------------------------------------------------------------------------\n   1. MEDICION ACTUAL Y ESTADO PERSISTENTE\n   --------------------------------------------------------------------------- */\n\n/* medicion del modo activo: posicion [mm] o fuerza [kN] */\nmed = x;\nif (modo>0.5) med = F;\n\n/* el estado llega como 12 ceros en la primera iteracion: rig>0 indica estado valido */\nif (sizeOfDim(S,0)>=12 && S[1]>0) {\n    x_ref=S[0]; rig=S[1]; F_pico=S[2]; integ=S[3]; sp_prev=S[4]; t_prev=S[5];\n    F_ref=S[6]; x_ref_rig=S[7]; x_inicio=S[8]; u_prev=S[9]; modo_prev=S[10]; causa_act=S[11];\n} else {\n    x_ref=x; rig=rig_ini; F_pico=0; integ=0; sp_prev=med; t_prev=tr;\n    F_ref=F; x_ref_rig=x; x_inicio=x; u_prev=0; modo_prev=modo; causa_act=0;\n}\n\ndt = tr - t_prev;\nif (dt<=0 || dt>1) dt = 0.02;   /* lectura de tiempo invalida: usa el periodo nominal */\n\nx_ref_ini = x_ref;   /* x_ref al empezar el paso (la proteccion de fuerza lo restituye) */\nprot = 0;\nst = stp;  f0 = f0p;  ts = tsp;\n\n/* ---------------------------------------------------------------------------\n   2. MAGNITUDES DERIVADAS Y LIMITES\n   --------------------------------------------------------------------------- */\n\n/* fuerza estimada por las presiones [kN] y corte por presiones (hoy desactivado) */\nF_pres = cFpA*pa - cFpB*pb;\nlim_pres = 0;\nif (prot_pres_on>0.5 && (pa>=pa_max || F_pres>=F_corte)) lim_pres = 1;\n\n/* velocidad de aproximacion [mm/min] y limite de fuerza fuera de ensayo [kN] */\nv_aprox = vjog;\nif (v_aprox<=0) v_aprox = 25;\nv_aprox = min(50,v_aprox);\n\nF_lib = abs(Flib);\nif (F_lib<=0) F_lib = 4;\nF_lib = max(0.2,min(50,F_lib));\n\n/* ---------------------------------------------------------------------------\n   3. INICIO DEL ENSAYO\n   El ensayo arranca en el flanco de subida de INICIAR (ini >= 5, inip < 5).\n   inio devuelve ini para que el diagrama lo realimente como inip.\n   --------------------------------------------------------------------------- */\ninio = ini;\n\n/* reinicio sin salto al iniciar o al cambiar el tipo de control */\nif ((ini>=5 && inip<5) || modo!=modo_prev) {\n    x_ref = x;\n    integ = 0;\n    sp_prev = med;\n}\n\n/* ---------------------------------------------------------------------------\n   4. GENERADOR DE CONSIGNA sp (maquina de estados)\n   --------------------------------------------------------------------------- */\nif (ini<5) {\n    /* FUERA DE ENSAYO: avance a v_aprox, retorno a v_retorno. Lento solo si se\n       avanza con compresion (F > frac_freno*F_lib); el retorno nunca se frena.\n       En fuerza, la consigna spm se limita a +-F_lib (o +-F_corte si sinprot). */\n    st = ST_REPOSO;\n    causa_act = CAU_NINGUNA;\n    if (modo>0.5) {\n        if (sinprot>0.5) {\n            dif = max(-F_corte,min(F_corte,spm)) - sp_prev;\n        } else {\n            dif = max(-F_lib,min(F_lib,spm)) - sp_prev;\n        }\n        vel_sp = v_des;\n        paso_sp = vel_sp*dt/60;\n        if (paso_sp<=0) paso_sp = 1e9;\n    } else {\n        dif = spm - sp_prev;\n        vel_sp = v_aprox;\n        if (dif<0) vel_sp = v_retorno;\n        if (sinprot<0.5 && dif>0 && F>frac_freno*F_lib) vel_sp = min(v_aprox,v_lenta);\n        paso_sp = vel_sp*dt/60;\n    }\n    /* la consigna sigue a spm con pendiente limitada a paso_sp por paso */\n    sp = sp_prev + max(-paso_sp,min(paso_sp,dif));\n} else {\n    /* EN ENSAYO */\n    if (inip<5) {\n        /* primer paso del ensayo: arranca la carga desde la medicion actual */\n        st = ST_CARGA;\n        f0 = med;\n        ts = t;\n        F_pico = 0;\n        F_ref = F;\n        x_ref_rig = x;\n        x_inicio = x;\n        causa_act = CAU_NINGUNA;\n    }\n    dif = lim - f0;\n    if (st==ST_CARGA) {\n        /* carga: rampa hacia lim */\n        sp = f0 + sign(dif)*abs(rate)*(t-ts)/60;\n        if (dif*(sp-lim)>=0) { sp=lim; st=ST_MANTIENE; ts=t; }\n    } else if (st==ST_MANTIENE) {\n        /* mantener lim durante tc segundos */\n        sp = lim;\n        if (t-ts>=tc) { st=ST_DESCARGA; ts=t; }\n    } else if (st==ST_DESCARGA) {\n        /* descarga: a v_retorno [mm/min] en desplazamiento, a v_des [kN/min] en fuerza */\n        vel_sp = v_des;\n        if (modo<0.5) vel_sp = v_retorno;\n        sp = lim - sign(dif)*vel_sp*(t-ts)/60;\n        if (dif*(f0-sp)>=0) { sp=f0; st=ST_RETORNO; ts=t; }\n    } else {\n        /* retorno/fin (4) o FALLA (5): consigna en el valor inicial */\n        sp = f0;\n    }\n}\n\n\n/* ---------------------------------------------------------------------------\n   5. RIGIDEZ ESTIMADA rig = dF/dx\n   En linea en todo momento salvo retorno y falla (reposo, aproximacion, carga,\n   mantenimiento y descarga, en ambos modos): asi el lazo de fuerza usa la\n   rigidez real.\n   --------------------------------------------------------------------------- */\ndF_min = dF_min_rig;\nif (ini>=5) dF_min = max(dF_min_rig,dF_min_rig*abs(lim-f0));\nif (st<=ST_DESCARGA && abs(F-F_ref)>dF_min && abs(x-x_ref_rig)>dx_min_rig) {\n    rig_nueva = (F-F_ref)/(x-x_ref_rig);\n    if (rig_nueva>rig_min) rig = rig + alfa_rig*(rig_nueva-rig);\n    F_ref = F;\n    x_ref_rig = x;\n}\nif (abs(x-x_ref_rig)>dx_sin_contacto) { F_ref=F; x_ref_rig=x; }   /* sin contacto: reinicia la referencia */\nrig = max(rig_min,min(rig_max,rig));\n\n\n/* ---------------------------------------------------------------------------\n   6. LAZO EXTERNO: consigna de posicion x_ref\n   --------------------------------------------------------------------------- */\nif (modo>0.5) {\n    /* control de fuerza */\n    if (st==ST_RETORNO) {\n        /* retorno a la posicion inicial x_inicio a v_retorno */\n        x_ref = x_ref + sign(x_inicio-x_ref)*min(abs(x_inicio-x_ref),v_retorno*dt/60);\n    } else if (st!=ST_FALLA) {\n        /* prealimentacion de la rampa + correccion normalizada por rigidez */\n        x_ref_prev = x_ref;\n        x_ref = x_ref + (sp-sp_prev)/rig + Kf*(sp-F)/rig*dt;\n        /* velocidad maxima del piston = v_aprox (evita embalarse sin contacto) */\n        if (st<=ST_DESCARGA) x_ref = x_ref_prev + max(-v_aprox*dt/60,min(v_aprox*dt/60,x_ref-x_ref_prev));\n    }\n} else {\n    /* control de desplazamiento */\n    if (st!=ST_FALLA) x_ref = sp;\n}\n\n\n/* ---------------------------------------------------------------------------\n   7. PROTECCION DE FUERZA FUERA DE ENSAYO\n   Con compresion F > F_lib no deja avanzar; retroceder (alejarse) siempre esta\n   permitido.\n   --------------------------------------------------------------------------- */\nif (st==ST_REPOSO && sinprot<0.5) {\n    if (F>F_lib) { x_ref=min(x_ref,x_ref_ini); integ=min(integ,0); prot=1; }\n    if (prot>0.5 && modo<0.5) sp = x_ref;\n}\n\n\n/* ---------------------------------------------------------------------------\n   8. DETECCION DE FALLA, LIMITES Y PARO DE EMERGENCIA\n   --------------------------------------------------------------------------- */\nif (st>=ST_CARGA && st<=ST_DESCARGA) {\n    F_pico = max(F_pico,F);\n    if (modo>0.5 && st<=ST_MANTIENE && F_pico>frac_pico_min*abs(lim) && F<(1-frac_caida)*F_pico) {\n        st=ST_FALLA; causa_act=CAU_CAIDA; x_ref=x;           /* caida de carga */\n    } else if (modo>0.5 && F>frac_sobre*abs(lim)) {\n        st=ST_FALLA; causa_act=CAU_SOBRECARGA; x_ref=x;      /* sobrecarga */\n    } else if (x>xlim+margen_xlim) {\n        st=ST_FALLA; causa_act=CAU_LIM_POS; x_ref=x;         /* limite de posicion */\n    }\n}\n/* limite del sistema: en ensayo se declara FALLA */\nif (st>=ST_CARGA && st<=ST_RETORNO && abs(F)>=F_corte) { st=ST_FALLA; causa_act=CAU_FCORTE;  x_ref=x; }\nif (st>=ST_CARGA && st<=ST_RETORNO && lim_pres>0.5)    { st=ST_FALLA; causa_act=CAU_PRESION; x_ref=x; }\nif (paro>0.5 && ini>=5)  { st=ST_FALLA; causa_act=CAU_PARO; }\nif (st==ST_FALLA) sp = med;\nif (modo>0.5) sp = max(-F_corte,min(F_corte,sp));   /* consigna de fuerza nunca sobre el corte */\n\n\n/* ---------------------------------------------------------------------------\n   9. LAZO INTERNO DE POSICION (PI con anti-windup) Y SEGURIDADES DE SALIDA\n   --------------------------------------------------------------------------- */\nx_ref = max(x-x_win,min(x+x_win,x_ref));\nerr = x_ref - x;\nu_pi = Kx*(err+integ/Tix);\nif (abs(u_pi)<u_max) integ = integ + err*dt;                 /* integra solo si no satura */\nu = max(-u_max,min(u_max,u_pi));\nu = max(u_prev-du_max*dt,min(u_prev+du_max*dt,u));           /* limite de variacion (V/s) */\n\n/* LIMITE DEL SISTEMA: desde F_corte no se permite empujar mas, en cualquier estado y modo */\nif (F>=F_corte)  { u=min(u,0); integ=min(integ,0); x_ref=min(x_ref,x); prot=1; }\nif (F<=-F_corte) { u=max(u,0); integ=max(integ,0); x_ref=max(x_ref,x); prot=1; }\n/* corte por presiones (solo si prot_pres_on = 1) */\nif (lim_pres>0.5) { u=min(u,0); integ=min(integ,0); x_ref=min(x_ref,x); prot=1; }\n/* PARO: 0 V y seguimiento, para que al soltarlo no haya salto */\nif (paro>0.5) { u=0; integ=0; x_ref=x; sp=med; }\n\n\n/* ---------------------------------------------------------------------------\n   10. INDICADORES PARA LA INTERFAZ\n   --------------------------------------------------------------------------- */\nprog = 0;\ntrest = 0;\nif (st==ST_MANTIENE) {\n    if (tc>0) prog = 100*min(1,(t-ts)/tc);\n    trest = max(0,tc-(t-ts));\n}\nif (st==ST_DESCARGA || st==ST_RETORNO) prog = 100;\nfalla = 0;\nif (st==ST_FALLA) falla = 1;\ncausa = causa_act;\nif (paro>0.5) { causa=CAU_PARO; falla=1; }   /* alarma de PARO tambien fuera de ensayo */\nFpko = F_pico;\n\n\n/* ---------------------------------------------------------------------------\n   11. ESTADO PARA EL SIGUIENTE PASO Y REGISTRO\n   --------------------------------------------------------------------------- */\nsp_prev = sp;\nu_prev = u;\nt_prev = tr;\nmodo_prev = modo;\n\nSo[0]=x_ref;  So[1]=rig;       So[2]=F_pico;  So[3]=integ;     So[4]=sp_prev; So[5]=t_prev;\nSo[6]=F_ref;  So[7]=x_ref_rig; So[8]=x_inicio; So[9]=u_prev;   So[10]=modo_prev; So[11]=causa_act;\nxspo = x_ref;\nkho = rig;\n\nLg[0]=t;    Lg[1]=st;   Lg[2]=sp;   Lg[3]=F;   Lg[4]=x;   Lg[5]=x_ref;\nLg[6]=u;    Lg[7]=rig;  Lg[8]=dt;   Lg[9]=falla; Lg[10]=causa; Lg[11]=prot;\nLg[12]=pa;  Lg[13]=pb;  Lg[14]=F_pres;\n\n\n/* ---------------------------------------------------------------------------\n   12. PROTECCION ANTE DATOS INVALIDOS\n   Lectura invalida del cDAQ (NaN en posicion o fuerza) o P incompleto: salida\n   0 V, FALLA en ensayo y reinicio del estado (So[1]=0 hace que el proximo paso\n   lo descarte).\n   --------------------------------------------------------------------------- */\nif (!(x==x) || !(F==F) || par_ok<0.5) {\n    u = 0;\n    falla = 1;\n    So[1] = 0;\n    if (st>=ST_CARGA && st<=ST_RETORNO) st = ST_FALLA;\n    Lg[6] = 0;\n    Lg[9] = 1;\n}"("ini"=w327, "lim"=w326, "rate"=w325, "tc"=w323, "t"=w322, "spm"=w321, "stp"=w324, "f0p"=w332, "tsp"=w330, "inip"=w328, "F"=w283, "x"=w285, "modo"=w317, "xlim"=w316, "S"=w318, "P"=w312, "paro"=w302, "tr"=w295, "vjog"="Vel. aproximacion (mm/min)", "Flib"="Fmax fuera de ensayo (kN)", "sinprot"=w289, "pa"=w281, "pb"=w280) -> ("sp"=w320:dbl, "st"=w294:dbl, "f0"=w333:dbl, "ts"=w331:dbl, "inio"=w329:dbl, "u"=w315:dbl, "So"=w319:dbl[], "xspo"=→"Consigna posicion interna (mm)":dbl, "kho"=→"Rigidez estimada (kN/mm)":dbl, "prog"=→"Progreso mantenimiento":dbl, "trest"=→"Tiempo restante carga (s)":dbl, "causa"=w300:dbl, "Fpko"=→"Carga maxima (kN)":dbl, "prot"=w297:dbl, "Lg"=w292:dbl[])  [unwired: 1 out]
    "Estado del ensayo" <- w294
    "Causa de la falla" <- w300
    "Lg log" <- w292
    n165 = feedback-in #5(w319) -> ()
    n166 = Bundle("Numeric"=w322, "mean"=w285, "mean"=w283, "mean"=w281, "mean"=w280, "sp"=w320) -> (w334:T6)  [unwired: 1 in]
    n167 = feedback-in #6(w294) -> ()
    n168 = feedback-in #7(w329) -> ()
    n169 = feedback-in #8(w333) -> ()
    n170 = feedback-in #9(w331) -> ()
    n171 = call-poly <vilib>:"DAQmx Write.vi"("task/channels in"=w364, "data"=w315, "error in"=w363) -> ("task out"=w366:refnum<k21>, "error out"=w365:errorcluster)  [unwired: 10 in, 1 out]
    n172 = Greater Than 0?(x=w300) -> (x > 0?=→"Falla":bool)
    n173 = Greater Than 0?(x=w297) -> (x > 0?=→"Proteccion de fuerza activa":bool)
    n174 = Greater Than 0?(x=w294) -> (x > 0?=w291:bool)
    n175 = case shown="True" w291 {
      tunnel: w292 -> [_ w378]
      frame False {
      }
      frame True {
        n176 = global read "GlobalesPrensa.vi" "ArchivoControl"() -> (w377:path)
        n177 = call-poly <vilib>:"Write Delimited Spreadsheet.vi"("file path (dialog if empty)"=w377, "format (%.3f)"="%.5f", "2D data"=dbl[][] [], "1D data"=w378, "append to file? (new file:F)"=TRUE, "error in (no error)"=errorcluster {"status"=FALSE, "code"=0, "source"=""}, "transpose? (no:F)"=FALSE, "delimiter (\\t)"="\t" ("delimiter (\\t)")) -> ()  [unwired: 6 in, 2 out]
      }
    }
    n178 = global write "GlobalesPrensa.vi" "Ensayando"(w291) -> ()
    n179 = call <vilib>:"Boolean Crossing PtByPt.vi"("input"=w291) -> ("crossing"=w293:bool)  [unwired: 2 in]
    n180 = case shown="True" w293 {
      frame False {
      }
      frame True {
        n181 = property on="Tenacidad en vigas" class="Ring (strict)"() -> ("RingText.Text"=w379:string)  [unwired: 2 in, 2 out]
        n182 = global write "GlobalesPrensa.vi" "InfoEnsayo"(w379) -> ()
      }
    }
    n183 = call <extravilib>:"Write.vi"("element"=w334) -> ("channel"=w349:T7)  [unwired: 1 out]
  }
  n184 = call <vilib>:"DAQmx Stop Task.vi"("task/channels in"=w63, "error in"=w61) -> ("task out"=w62:refnum<k21>, "error out"=w60:errorcluster)  [unwired: 12 in]
  n185 = call <vilib>:"DAQmx Stop Task.vi"("task/channels in"=w89, "error in"=w88) -> ("task out"=w90:refnum<k21>, "error out"=w91:errorcluster)  [unwired: 12 in]
  n186 = while {
    tunnel: [w386] -> w51
    tunnel: w68 -> [w407]
    tunnel: w6 -> [w427]
    shift-right: [w402] -> _
    shift-left: dbl[] [] -> [w404]
    shift-right: [w401] -> _
    shift-left: dbl[] [] -> [w403]
    stop <- w426 stop-if-true
    # "Bloqueo: APLICAR NORMA solo actua en reposo (0) o falla (5)"
    n187 = call <extravilib>:"Read.vi"("channel"=w427) -> ("element"=w426:bool)  [unwired: 1 in, 1 out]
    n188 = call <extravilib>:"Read.vi"("channel"=w407) -> ("element"=w416:T9)  [unwired: 1 in, 1 out]
    n189 = Unbundle(w416) -> ("Numeric"=→"Tiempo (s)":dbl, w405:dbl, w406:dbl, →"Presión A (bar)":dbl, →"Presión B (bar)":dbl, "Limite fuerza (kN)"=w412:dbl)
    "Fuerza actual (KN)" <- w406
    "Posicion actual (mm)" <- w405
    "Vertical Progress Bar" <- w405
    n190 = Insert Into Array(array=w404, new element=w405) -> (w402:dbl[])  [unwired: 1 in]
    n191 = Insert Into Array(array=w403, new element=w406) -> (w401:dbl[])  [unwired: 1 in]
    n192 = case shown="1" "Tipo ensayos" {
      tunnel: [w439 w449] -> w396
      frame 0, Default {
        n193 = property on="Flexotracción en losas" class="Ring (strict)"("Visible"=TRUE) -> ()  [unwired: 2 in, 2 out]
        n194 = property on="Velocidad norma (mm/min)" class="DigNum (strict)"("Visible"=TRUE) -> ()  [unwired: 2 in, 2 out]
        n195 = property on="Tenacidad en vigas" class="Ring (strict)"("Visible"=FALSE) -> ()  [unwired: 2 in, 2 out]
        n196 = property on="Velocidad norma (mm/min)  2" class="Str"("Visible"=FALSE) -> ()  [unwired: 2 in, 2 out]
        n197 = case shown="2" "Flexotracción en losas" {
          tunnel: [1.5 4.0 1.0 1.0] -> w439
          frame 0, Default {
          }
          frame 3 {
          }
          frame 2 {
          }
          frame 1 {
          }
        }
        "Velocidad norma (mm/min)" <- w439
      }
      frame 1 {
        n198 = property on="Tenacidad en vigas" class="Ring (strict)"("Visible"=TRUE) -> ()  [unwired: 2 in, 2 out]
        n199 = property on="Velocidad norma (mm/min)" class="DigNum (strict)"("Visible"=FALSE) -> ()  [unwired: 2 in, 2 out]
        n200 = property on="Velocidad norma (mm/min)  2" class="Str"("Visible"=TRUE) -> ()  [unwired: 2 in, 2 out]
        n201 = property on="Flexotracción en losas" class="Ring (strict)"("Visible"=FALSE) -> ()  [unwired: 2 in, 2 out]
        n202 = case shown="0, Default" "Tenacidad en vigas" {
          tunnel: ["0.05 - 0.1" "0.06 - 0.12" "0.1" "0.5 ± 0.05" "0.25"] -> w450
          frame 0, Default {
          }
          frame 1 {
          }
          frame 3 {
          }
          frame 4 {
          }
          frame 2 {
          }
        }
        "Velocidad norma (mm/min)  2" <- w450
        n203 = Fract/Exp String To Number(string=w450) -> (number=w449:dbl)  [unwired: 3 in, 1 out]
      }
    }
    n204 = Bundle(w402, w401) -> (→"fuerza desplazamiento":cluster{dbl[], dbl[]})  [unwired: 1 in]
    n205 = Wait (ms)(milliseconds to wait=u32 100) -> ()  [unwired: 1 out]
    n206 = local read "Estado del ensayo"() -> (w395:dbl)
    n207 = case shown="0, Default" "Tipo control" {
      tunnel: [w434 w438] -> w411
      tunnel: w406 -> [w433 w438]
      tunnel: w405 -> [w434 w437]
      frame 0, Default {
        n208 = local write "Fuerza deseada (kN)"(w433) -> ()
        n209 = property on="Fuerza deseada (kN)" class="DigNum (strict)"("DisabledEnum"=T8."Disabled" ("Disabled")) -> ()  [unwired: 2 in, 2 out]
        n210 = property on="Posicion deseada (mm)" class="Slide (strict)"("DisabledEnum"=T8."Enabled" ("Disabled")) -> ()  [unwired: 2 in, 2 out]
      }
      frame 1 {
        n211 = local write "Posicion deseada (mm)"(w437) -> ()
        n212 = property on="Fuerza deseada (kN)" class="DigNum (strict)"("DisabledEnum"=T8."Enabled" ("Disabled")) -> ()  [unwired: 2 in, 2 out]
        n213 = property on="Posicion deseada (mm)" class="Slide (strict)"("DisabledEnum"=T8."Disabled" ("Disabled")) -> ()  [unwired: 2 in, 2 out]
      }
    }
    n214 = Equal To 0?(x="Tipo control") -> (x = 0?=w399:bool)
    n215 = Not Equal To 0?(x="Tipo control") -> (x != 0?=w398:bool)
    n216 = Select(t=T8."Disabled" ("Disabled"), s="Iniciar ensayo", f=T8."Enabled" ("Disabled")) -> (s? t:f=w408:T8)
    n217 = In Range and Coerce(upper limit=4.5, x=w395, lower limit=0.5) -> (In Range?=w392:bool)  [unwired: 1 out]
    n218 = property on="Limite fuerza (kN)" class="DigNum (strict)"("DisabledEnum"=w408) -> ()  [unwired: 2 in, 2 out]
    n219 = property on="Rampa (kN/min)" class="DigNum (strict)"("DisabledEnum"=w408) -> ()  [unwired: 2 in, 2 out]
    n220 = property on="Rampa (mm/min)" class="DigNum (strict)"("Visible"=w399) -> ()  [unwired: 2 in, 2 out]
    n221 = property on="Limite fuerza (kN)" class="DigNum (strict)"("Visible"=w398) -> ()  [unwired: 2 in, 2 out]
    n222 = property on="Rampa (kN/min)" class="DigNum (strict)"("Visible"=w398) -> ()  [unwired: 2 in, 2 out]
    n223 = property on="Fuerza deseada (kN)" class="DigNum (strict)"("DisabledEnum"=w408) -> ()  [unwired: 2 in, 2 out]
    n224 = property on="Posicion deseada (mm)" class="Slide (strict)"("DisabledEnum"=w408) -> ()  [unwired: 2 in, 2 out]
    n225 = property on="Tiempo carga (s)" class="DigNum (strict)"("DisabledEnum"=w408) -> ()  [unwired: 2 in, 2 out]
    n226 = property on="Limite posicion (mm)" class="DigNum (strict)"("DisabledEnum"=w408) -> ()  [unwired: 2 in, 2 out]
    n227 = Not(x=w392) -> (.not. x?=w391:bool)
    n228 = And(x="Aplicar velocidad de norma", y=w391) -> (x .and. y?=w389:bool)
    n229 = case shown="False" w389 {
      tunnel: w396 -> [_ w429]
      frame False {
      }
      frame True {
        n230 = local write "Rampa (mm/min)"(w429) -> ()
        n231 = local write "Tipo control"(enum16{"Desplazamiento", "Fuerza"}."Desplazamiento" ("Tipo control")) -> ()
      }
    }
    n232 = Bundle("Rampa (mm/min)"="Rampa (mm/min)", "Rampa (kN/min)"="Rampa (kN/min)", "Limite posicion (mm)"="Limite posicion (mm)", "Limite fuerza (kN)"="Limite fuerza (kN)", "Posicion deseada (mm)"="Posicion deseada (mm)", "Fuerza deseada (kN)"="Fuerza deseada (kN)", "Tiempo carga (s)"="Tiempo carga (s)", "Iniciar ensayo"="Iniciar ensayo", "Tipo control"="Tipo control") -> (w387:T5)  [unwired: 1 in]
    n233 = Merge Signals(w412, w411) -> (→"control signals":dynamicdata)
    n234 = call <extravilib>:"Write.vi"("element"=w387) -> ("channel"=w386:T10)  [unwired: 1 out]
  }
  n235 = call <vilib>:"DAQmx Clear Task.vi"("task in"=w62, "error in"=w60) -> ("error out"=w84:errorcluster)  [unwired: 13 in]
  n236 = call <vilib>:"DAQmx Clear Task.vi"("task in"=w90, "error in"=w91) -> ("error out"=w85:errorcluster)  [unwired: 13 in]
  n237 = call <vilib>:"Simple Error Handler.vi"("error in (no error)"=w84) -> ()  [unwired: 4 in, 5 out]
  n238 = call <vilib>:"Simple Error Handler.vi"("error in (no error)"=w85) -> ()  [unwired: 4 in, 5 out]
